vi "Init Vecto.vi"(8 "error in (no error)":errorcluster, 11 "Volatus Core in":refnum<class "Volatus Core.lvclass">) -> (0 "error out":errorcluster, 3 "Volatus Core out":refnum<class "Volatus Core.lvclass">)   [LabVIEW 2020, in "Volatus.lvlib" / "Volatus Core.lvclass"]
uses:
  Volatus Core.lvclass
  C:/dev/lv20CE/relink/lv-volatus/Volatus/Module/Module.lvclass
  lv-vecto/Vecto/Event Level.ctl
  lv-vecto/Vecto/Init Implementations.ctl
  lv-vecto/Vecto/EventLogHandler/EventLogHandler.lvclass
  Volatus Core.lvclass/Volatus Core.ctl
  Module/Module.lvclass/Module.ctl
  VectoEventBridge/VectoEventBridge.lvclass
  C:/dev/lv20CE/relink/lv-vecto/Vecto/EventLogHandler/EventLogHandler.lvclass
  Module/Module.lvclass
  lv-vecto/Vecto/Vecto/Vecto.lvclass
  lv-vecto/Vecto/Vecto.lvlib
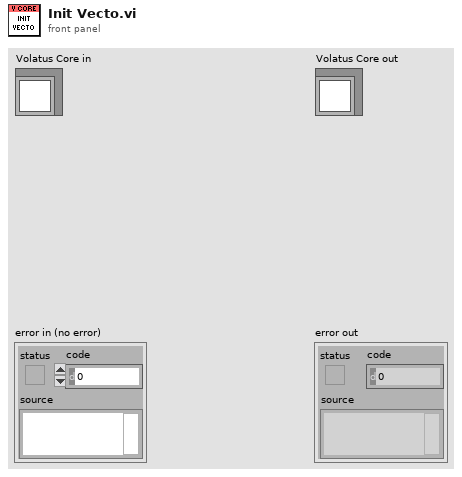
[diagram p1: front panel]
types:
  T1 = typedef "Vecto.lvlib/Init Implementations.ctl" = cluster{"EventLogger":refnum<class "EventLogHandler.lvclass">}
  T2 = typedef "Vecto.lvlib/Event Level.ctl" = enum16{"Debug", "Info", "Warning", "Error"}
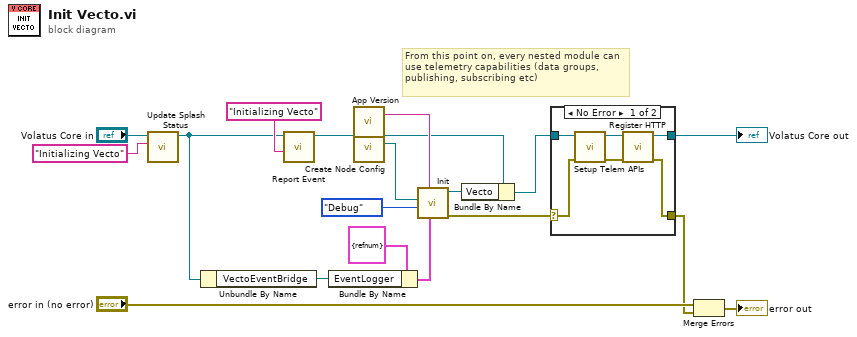
[diagram p0: block diagram]
diagram:
  # "From this point on, every nested module can use telemetry capabilities (data groups, publishing, subscribing etc)"
  n1 = call "Update Splash Status.vi"("Status"="Initializing Vecto", "Volatus Core in"="Volatus Core in") -> ("Volatus Core out"=w2:refnum<class "Volatus Core.lvclass">)  [unwired: 8 in, 1 out]
  n2 = Unbundle By Name(w2) -> ("VectoEventBridge"=w13:refnum<class "VectoEventBridge.lvclass">)
  n3 = call "Report Event.vi"("Message"="Initializing Vecto", "Module in"=w2) -> ("Module out"=w5:refnum<class "Volatus Core.lvclass">)  [unwired: 8 in, 1 out]
  n4 = Bundle By Name(cluster=T1 {"EventLogger"=refnum} ("Init Implementations"), "EventLogger"=w13) -> (w15:T1)
  n5 = call "App Version.vi"() -> ("App Version"=w12:string)  [unwired: 3 in]
  n6 = call "Create Node Config.vi"("Volatus Core in"=w5) -> ("Node"=w17:refnum<class "Node Config.lvclass">, "Volatus Core out"=w3:refnum<class "Volatus Core.lvclass">)  [unwired: 8 in, 1 out]
  n7 = call "Init.vi"("Init Implementations"=w15, "App Version"=w12, "Minimum Event Level (Info)"=Event_Level."Debug", "Node"=w17) -> ("error out"=w8:errorcluster, "Vecto out"=w10:refnum<class "Vecto.lvclass">)  [unwired: 6 in]
  n8 = Bundle By Name(cluster=w3, "Vecto"=w10) -> (w11:refnum<class "Volatus Core.lvclass">)
  n9 = case shown="No Error" w8 {
    selector: w8 -> [w24 w26]
    tunnel: w11 -> [w25 w27]
    tunnel: [w20 w27] -> w9
    tunnel: [w22 w26] -> w6
    frame No Error {
      n10 = call "Setup Telem APIs.vi"("error in (no error)"=w24, "Volatus Core in"=w25) -> ("error out"=w23:errorcluster, "Volatus Core out"=w21:refnum<class "Volatus Core.lvclass">)  [unwired: 8 in]
      n11 = call "Register HTTP.vi"("error in (no error)"=w23, "Volatus Core in"=w21) -> ("error out"=w22:errorcluster, "Volatus Core out"=w20:refnum<class "Volatus Core.lvclass">)  [unwired: 8 in]
    }
    frame Error {
    }
  }
  "Volatus Core out" <- w9
  n12 = Merge Errors("error in (no error)", w6) -> (→"error out":errorcluster)
